vi "setUp.vi"(8 "error in (no error)":errorcluster, 11 "reference in":refnum<class "EM1000 Turn Table.lvclass">) -> (0 "error out":errorcluster, 3 "reference out":refnum<class "EM1000 Turn Table.lvclass">)   [LabVIEW 2020, in "EM1000 Turn Table.lvclass"]
doc: "setUp runs prior to the test method during test execution. Use this method to initialize any object data required by your tests."
uses:
  EM1000 Turn Table.lvclass
  EM1000 Turn Table.lvclass/EM1000 Turn Table.ctl
  <vilib>/addons/_JKI Toolkits/VI Tester/TestCase.llb/TestCase.lvclass
  AUDIX EM1000.lvclass
  C:/Program Files (x86)/National Instruments/LabVIEW 2020/vi.lib/addons/_JKI Toolkits/VI Tester/TestCase.llb/TestCase.lvclass
  C:/_Git_Repo/fcc_Part15/Device Class/AUDIX EM1000/Test Code/EM1000 Turn Table/EM1000 Turn Table.lvclass
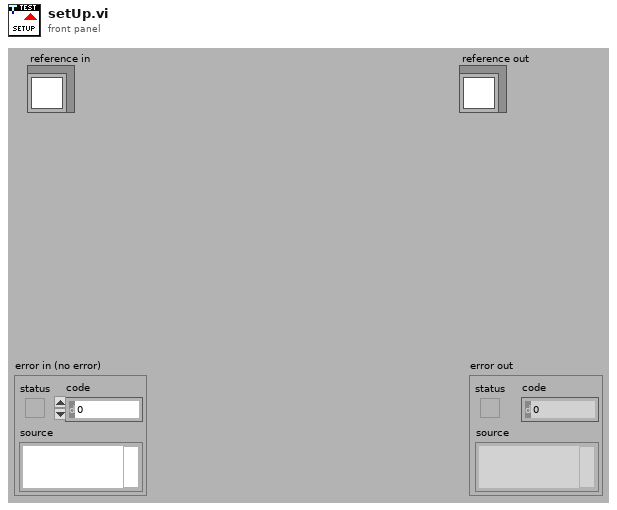
[diagram p1: front panel]
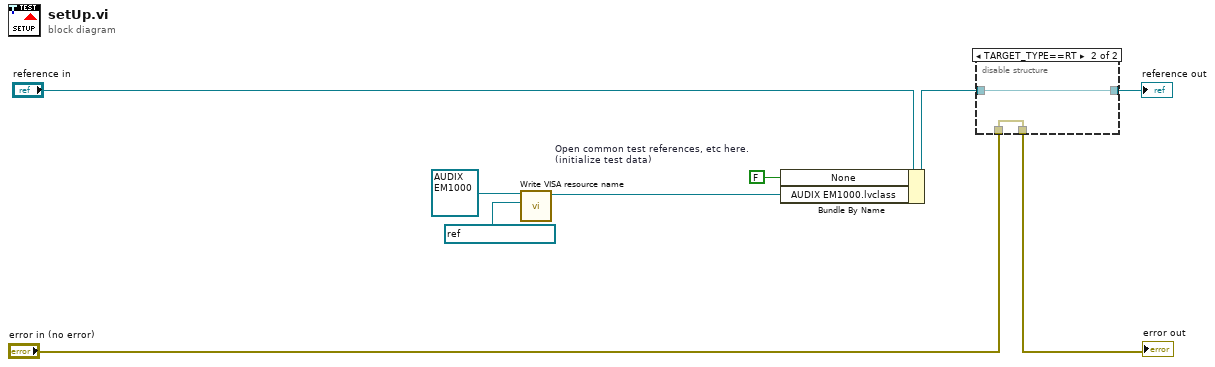
[diagram p0: block diagram]
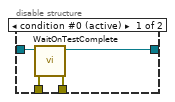
[diagram p2: hidden frame]
diagram:
  w4 = FALSE  # Open common test references, etc here. (initialize test data)
  n1 = call "Write VISA resource name.vi"("VISA resource name"=refnum<visa-resource-name> "GPIB0::5::INSTR", "AUDIX EM1000 in"=refnum<class "AUDIX EM1000.lvclass"> refnum ("AUDIX EM1000.lvclass")) -> ("AUDIX EM1000 out"=w1:refnum<class "AUDIX EM1000.lvclass">)  [unwired: 8 in, 1 out]
  n2 = Bundle By Name(cluster="reference in", "None"=w4, "AUDIX EM1000.lvclass"=w1) -> (w5:refnum<class "EM1000 Turn Table.lvclass">)
  n3 = disable-structure shown="TARGET_TYPE==RT" {
    disable-tunnel: "error in (no error)" -> [w13 w14]
    disable-tunnel: [w12 w14] -> w8
    disable-tunnel: [w11 w15] -> w6
    disable-tunnel: w5 -> [w10 w15]
    frame condition #0 (active) {
      n4 = call <vilib>:"WaitOnTestComplete.vi"("error in (no error)"=w13, "TestCase in"=w10) -> ("error out"=w12:errorcluster, "TestCase out"=w11:refnum<class "EM1000 Turn Table.lvclass">)  [unwired: 8 in]
    }
    frame condition #1 {
    }
  }
  "error out" <- w8
  "reference out" <- w6
